vi "Host_Lookup.vi"(10 "Key":u16, 11 "Table":string) -> (3 "Text":string)   [LabVIEW 2018]
doc: "Use this template to build a VI to use as a subVI."
panel:
  # "說明：代碼查文字，表格格式：換行 + 代碼 = 文字。從 13_PL\nC 複製。"
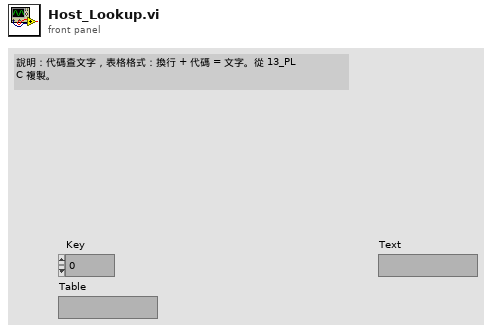
[diagram p1: front panel]
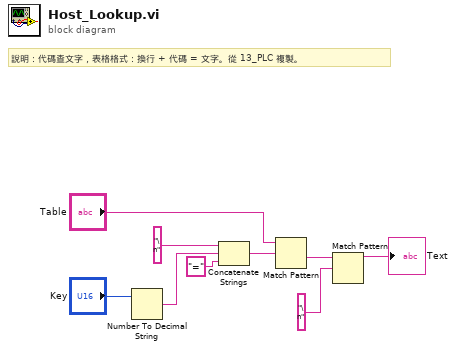
[diagram p0: block diagram]
diagram:
  # "說明：代碼查文字，表格格式：換行 + 代碼 = 文字。從 13_PLC 複製。"
  n1 = Number To Decimal String(number="Key") -> (decimal integer string=w7:string)  [unwired: 1 in]
  n2 = Concatenate Strings("\n", w7, "=") -> (w4:string)
  n3 = Match Pattern(string="Table", regular expression=w4) -> (after substring=w3:string)  [unwired: 1 in, 3 out]
  n4 = Match Pattern(string=w3, regular expression="\n") -> (before substring=→"Text":string)  [unwired: 1 in, 3 out]
